vi "Get String Indicator Reference.vi"(11 "error in (no error)":errorcluster) -> (4 "String":refnum<vi>, 6 "vi reference":refnum<vi>, 15 "error out":errorcluster)   [LabVIEW 2021, in "Migrator.lvlib"]
uses:
  Migrator.lvlib
  Path Functions/Path Functions.lvlib
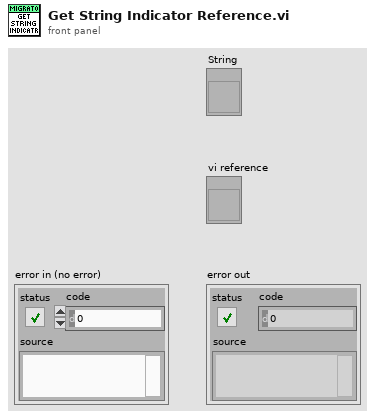
[diagram p1: front panel]
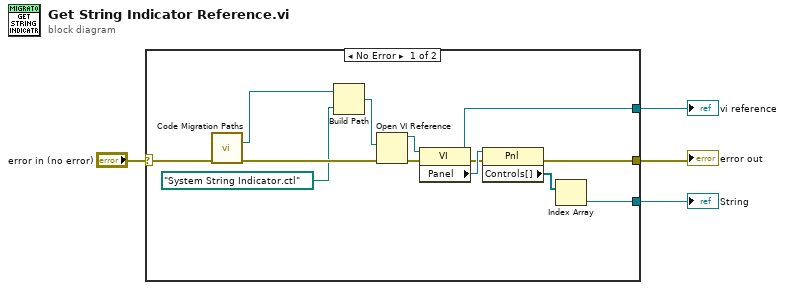
[diagram p0: block diagram]
diagram:
  n1 = case shown="No Error" "error in (no error)" {
    selector: "error in (no error)" -> [w8 w18]
    tunnel: [w9 _] -> w4
    tunnel: [w7 w18] -> w2
    tunnel: [w6 _] -> w1
    frame No Error {
      n2 = call "Code Migration Paths.vi"("error in (no error)"=w8) -> ("IO Controls"=w17:path, "error out"=w13:errorcluster)  [unwired: 6 in, 7 out]
      n3 = Build Path(base path=w17, name or relative path=path "System String Indicator.ctl") -> (appended path=w16:path)
      n4 = Open VI Reference(vi path=w16, error in (no error)=w13) -> (vi reference=w10:refnum<vi>, error out=w12:errorcluster)  [unwired: 4 in]
      n5 = property class="VI"(reference=w10, error in=w12) -> (reference out=w6:refnum<vi>, error out=w11:errorcluster, "Panel"=w15:refnum<vi>)
      n6 = property class="Pnl"(reference=w15, error in=w11) -> (error out=w7:errorcluster, "Controls[]"=w14:refnum<vi>[])  [unwired: 1 out]
      n7 = Index Array(array=w14) -> (element=w9:refnum<vi>)  [unwired: 1 in]
    }
    frame Error {
    }
  }
  "String" <- w4
  "error out" <- w2
  "vi reference" <- w1
